vi "Relink Save.vi"() -> ()   [LabVIEW 2020]
doc: "Dev helper for moving VIs: opens every VI listed in the preload file (one path per line) and keeps it in memory, then opens every VI in the items file from its NEW location and saves it, so LabVIEW links its subVIs to the preloaded VIs of the same name and stores the new relative paths. Move the files first (git mv), list their callees as preload. Returns the error code per item; closes everything at the end."
panel:
  out "error out":errorcluster
  out "codes":i32[](array[numeric])
  out "preload codes":i32[](array[numeric])
  in  "items file":path
  in  "preload file":path
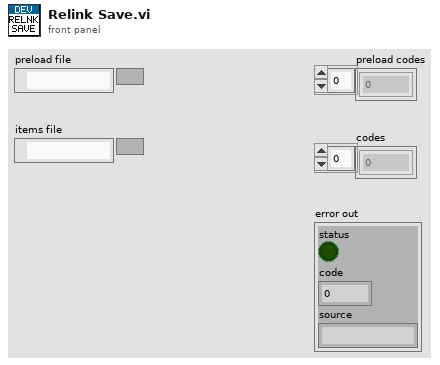
[diagram p1: front panel]
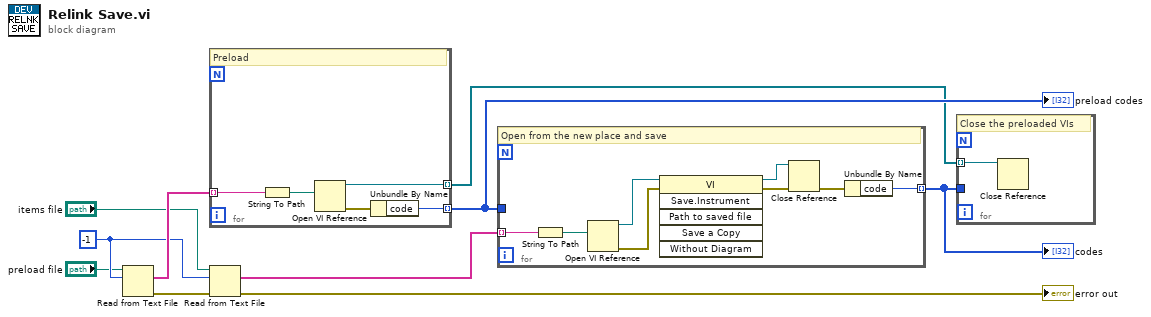
[diagram p0: block diagram]
diagram:
  w3 = -1
  n1 = Read from Text File(file (use dialog)="preload file", count=w3) -> (text=w4:string[], error out=w5:errorcluster)  [unwired: 2 in, 2 out]
  n2 = for {
    tunnel: w4 -> [w11] mode=indexing
    tunnel: [w13] -> w6 mode=indexing
    tunnel: [w15] -> w7 mode=indexing
    # "Preload"
    n3 = String To Path(string=w11) -> (path=w12:path)
    n4 = Open VI Reference(vi path=w12) -> (vi reference=w13:refnum<vi>, error out=w14:errorcluster)  [unwired: 5 in]
    n5 = Unbundle By Name(w14) -> ("code"=w15:i32)
  }
  "preload codes" <- w7
  n6 = Read from Text File(file (use dialog)="items file", count=w3, error in=w5) -> (text=w8:string[], error out=→"error out":errorcluster)  [unwired: 1 in, 2 out]
  n7 = for {
    tunnel: w8 -> [w16] mode=indexing
    tunnel: w7 -> [_]
    tunnel: [w23] -> w10 mode=indexing
    # "Open from the new place and save"
    n8 = String To Path(string=w16) -> (path=w17:path)
    n9 = Open VI Reference(vi path=w17) -> (vi reference=w18:refnum<vi>, error out=w19:errorcluster)  [unwired: 5 in]
    n10 = invoke class="VI" method="Save.Instrument"(reference=w18, error in=w19) -> (reference out=w20:refnum<vi>, error out=w21:errorcluster)  [unwired: 4 in, 4 out]
    n11 = Close Reference(reference=w20, error in (no error)=w21) -> (error out=w22:errorcluster)
    n12 = Unbundle By Name(w22) -> ("code"=w23:i32)
  }
  "codes" <- w10
  n13 = for {
    tunnel: w6 -> [w24] mode=indexing
    tunnel: w10 -> [_]
    # "Close the preloaded VIs"
    n14 = Close Reference(reference=w24) -> ()  [unwired: 1 in, 1 out]
  }
